vi "OpenG Conditiional Auto-Indexing Tunnel template.vi"() -> ()   [LabVIEW 2012]
uses:
  OpenG Reverse 2D Array/OpenG Reverse 2D Array.xnode
panel:
  in  "Elements to keep":bool[](array[boolean])
  in  "Array in":variant[](array[variant])
  out "Filtered Array out":variant[](array[variant])
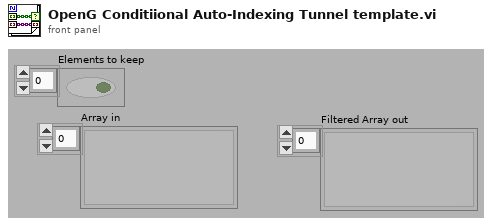
[diagram p1: front panel]
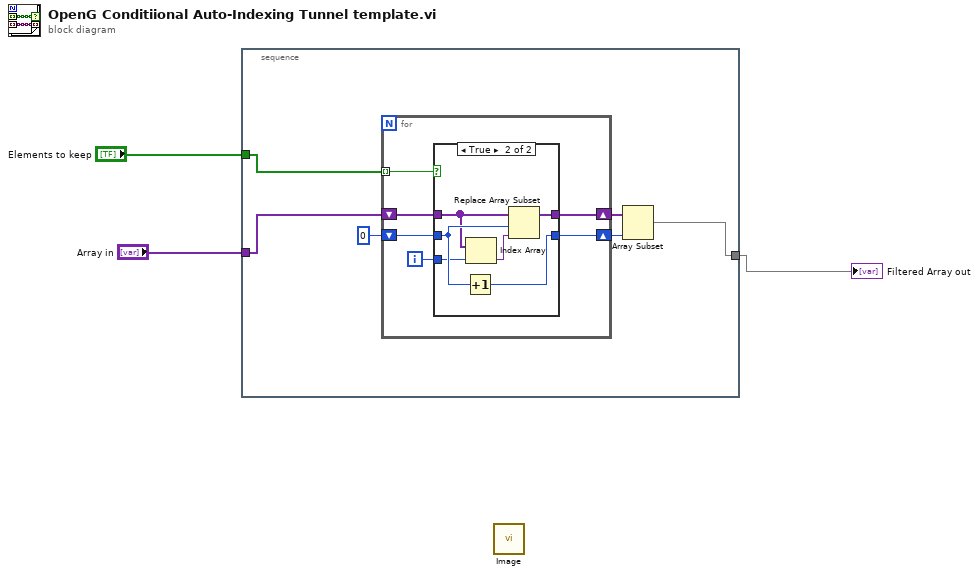
[diagram p0: block diagram]
diagram:
  n1 = stacked-sequence {
    tunnel: [w4] -> w1
    tunnel: "Array in" -> [w5]
    tunnel: "Elements to keep" -> [w6]
    frame #0 {
      n2 = for {
        shift-right: [w13] -> w9
        shift-left: 0 -> [w14]
        shift-right: [w12] -> w8
        shift-left: w5 -> [w15]
        tunnel: w6 -> [w11] mode=indexing
        i -> [w10]
        n3 = case shown="True" w11 {
          tunnel: w15 -> [w16 w20]
          tunnel: w14 -> [w17 w21]
          tunnel: [w17 w23] -> w13
          tunnel: [w16 w22] -> w12
          tunnel: w10 -> [_ w18]
          frame False {
          }
          frame True {
            n4 = Increment(x=w21) -> (x+1=w23:i32)
            n5 = Index Array(array=w20, index=w18) -> (element=w19:variant)
            n6 = Replace Array Subset(array=w20, new element=w19, index=w21) -> (w22:variant[])
          }
        }
      }
      n7 = Array Subset(array=w8, length=w9) -> (w4:variant[])  [unwired: 1 in]
    }
  }
  "Filtered Array out" <- w1
  n8 = call "Image.vi"() -> ()  [unwired: 2 in, 2 out]
